vi "State Callers.vi"(8 "synchronization":refnum<class "synchronization.lvclass">, 9 "Callers":T2, 10 "State":string, 11 "Calling VI Details":T1) -> (0 "error out":errorcluster)   [LabVIEW 2020]
uses:
  JKI State Machine API/source/Support/State Calls Array.ctl
  JKI State Machine API/source/Support/State Call Cluster.ctl
  JKI State Machine API/source/JKI SM/JKI SM.lvclass/JKI SM.ctl
  <userlib>/_OpenG.lib/error/error.llb/Filter Error Codes (Array)__ogtk.vi
  <vilib>/regexp/Match Regular Expression.xnode
  JKI State Machine API/source/JKI SM/JKI SM.lvclass
  <userlib>/_OpenG.lib/error/error.llb/openg_error.lvlib
  synchronization/synchronization.lvclass
panel:
  in  "Listbox":i32(listbox)
  in  "OK":bool
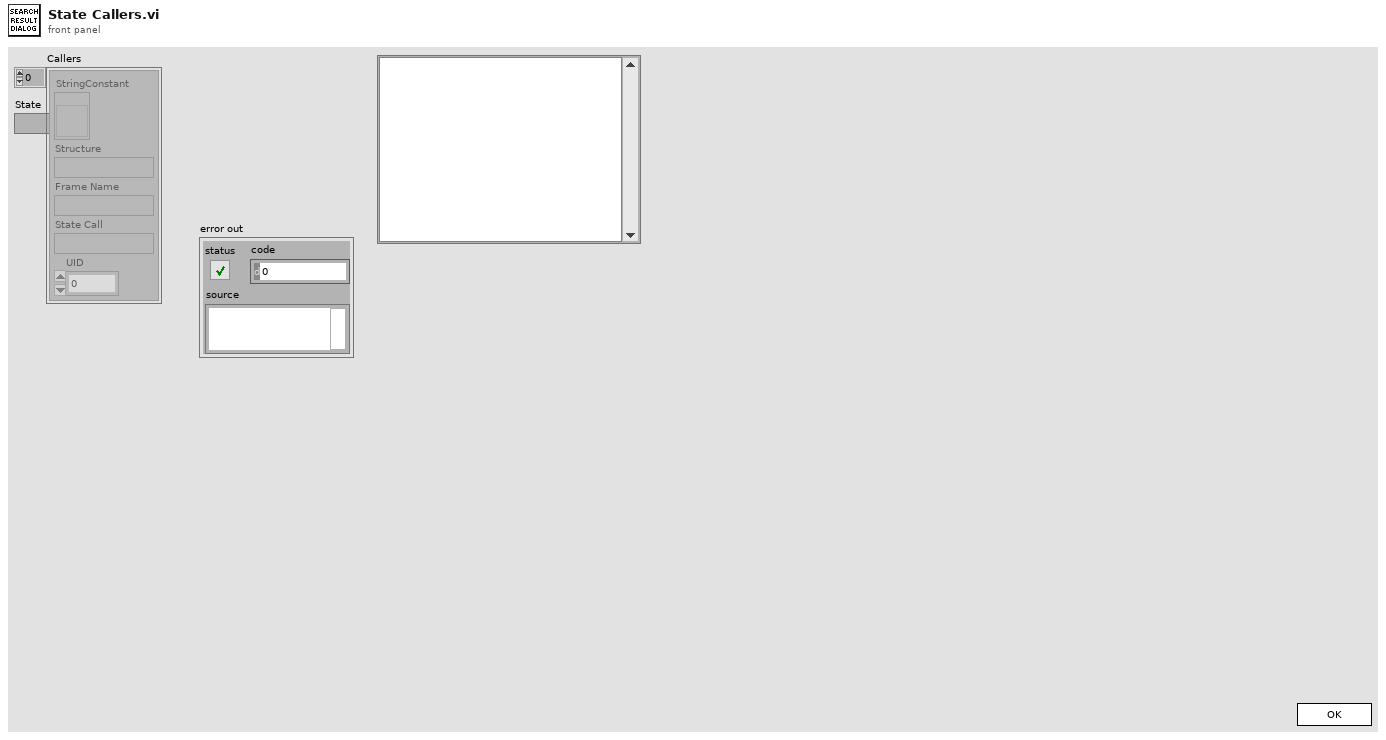
[diagram p1: front panel]
types:
  T1 = cluster{"App.ContextName":string, "VI.Name":string, "Object UID":i32}
  T2 = typedef "State Calls Array.ctl" = T3[]
  T3 = typedef "State Call Cluster.ctl" = cluster{"StringConstant":refnum<vi>, "Structure":string, "Frame Name":string, "State Call":string, "UID":i32}
  T4 = enum32{"Invalid", "Standard", "Closed", "Hidden", "Minimized", "Maximized"}
  T5 = enum32{"invalid app kind", "Development System", "Run Time System", "Student Edition", "Embedded LabVIEW", "Evaluation", "Custom"}
  T6 = enum32{"Invalid", "Default", "Floating", "Floating/Auto-Hide", "Modal"}
  T7 = cluster{"Core":cluster{"Current VI Reference":refnum<vi>, "Close Panel on Exit?":bool}, "Your Boolean data":bool, "Your string data":string, "State":string, "JKI SM out":refnum<class "JKI SM.lvclass">, "Callers":T2, "Application":refnum<vi>, "Owning VI":refnum<vi>}
  T8 = typedef "LVPoint32TypeDef.ctl" = cluster{"Horizontal":i32, "Vertical":i32}
  T9 = cluster{"Shift":bool, "Ctrl":bool, "Alt":bool, "Cmd":bool, "Opt":bool}
  T10 = cluster{"StringConstant":refnum<vi>, "Structure":string, "Frame Name":string, "State Call":string, "UID":dbl}[]
  T11 = cluster{"Current VI Reference":refnum<vi>, "Close Panel on Exit?":bool}
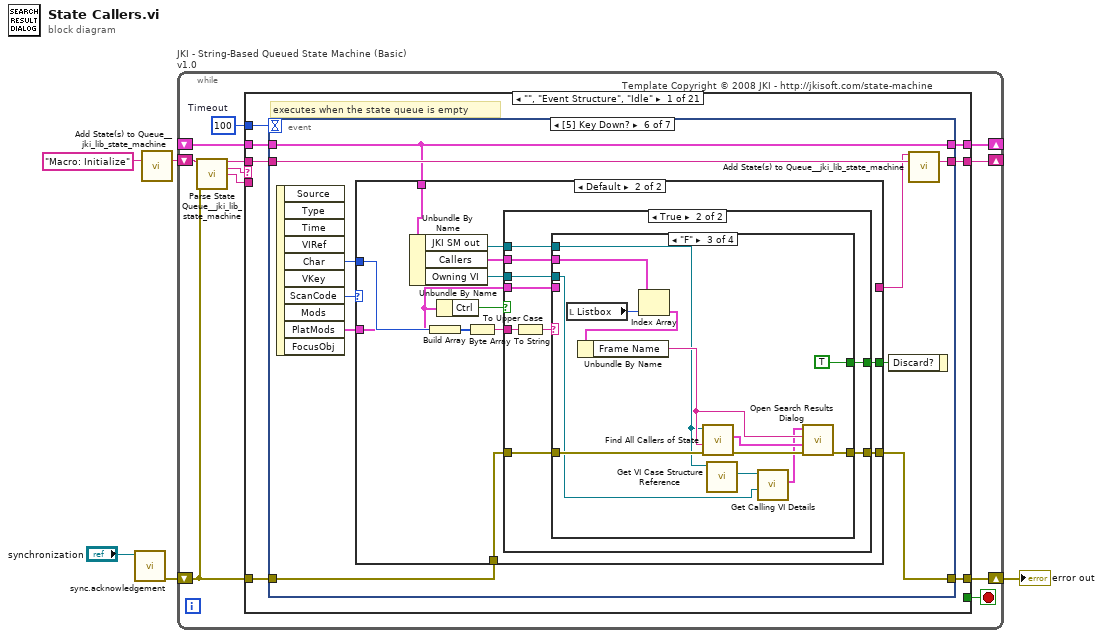
[diagram p0: block diagram]
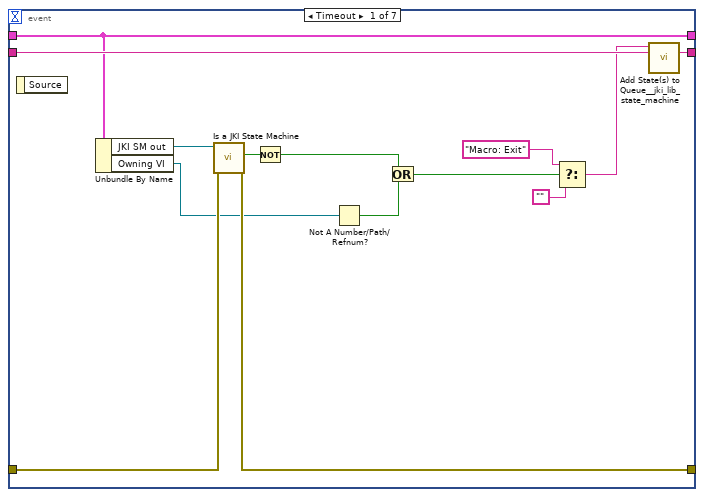
[diagram p2: hidden frame]
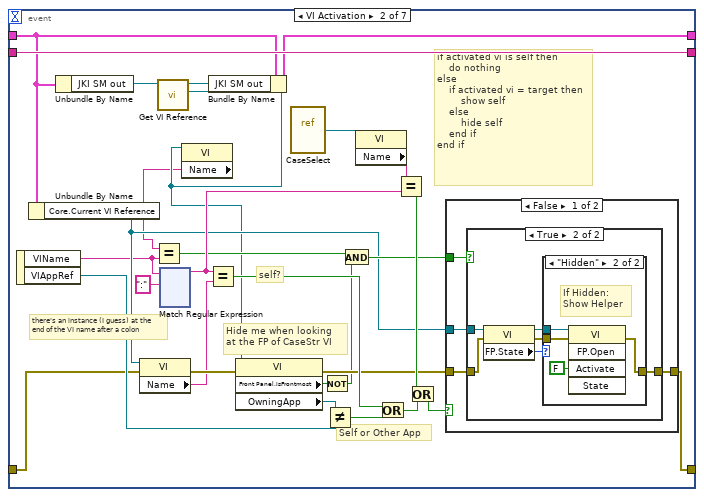
[diagram p3: hidden frame]
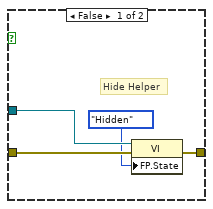
[diagram p4: hidden frame]
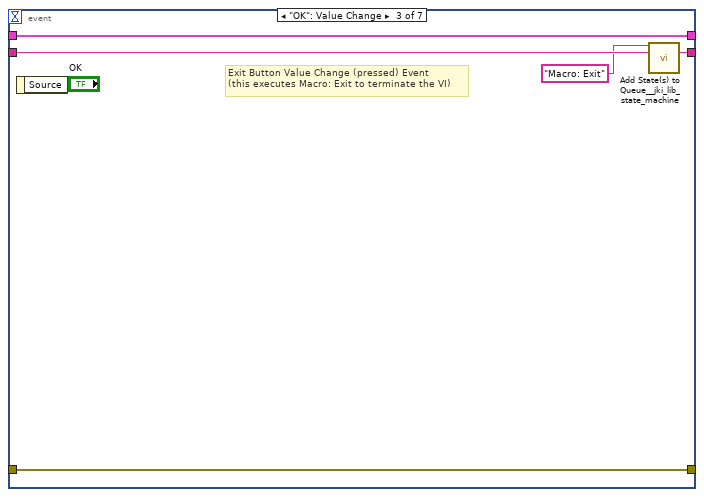
[diagram p7: hidden frame]
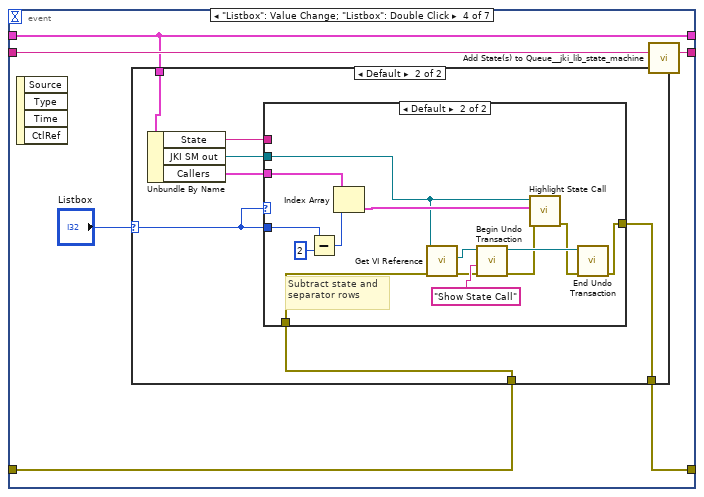
[diagram p8: hidden frame]
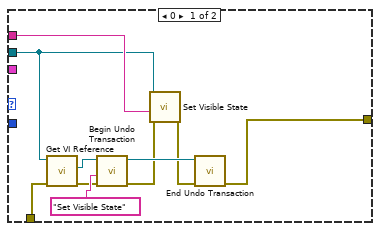
[diagram p10: hidden frame]
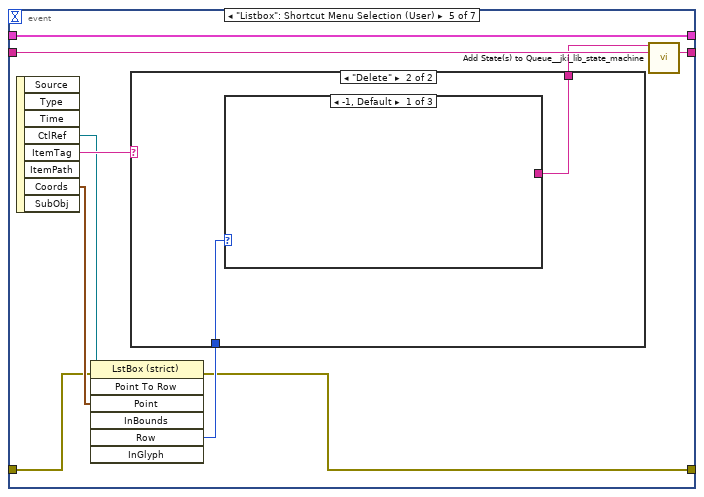
[diagram p11: hidden frame]
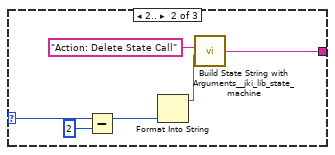
[diagram p13: hidden frame]
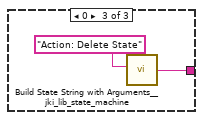
[diagram p14: hidden frame]
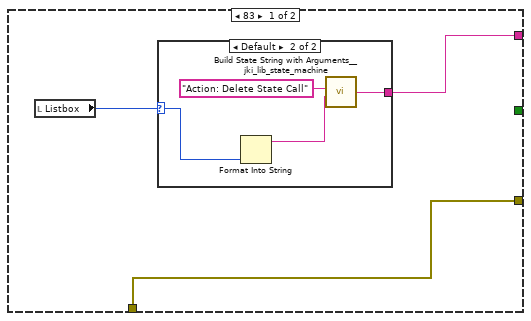
[diagram p15: hidden frame]
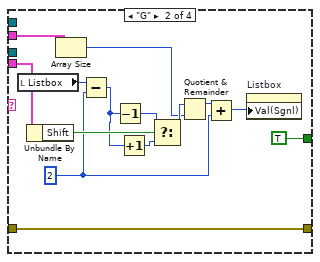
[diagram p19: hidden frame]
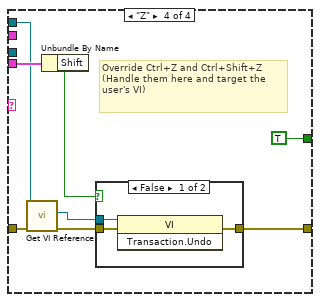
[diagram p20: hidden frame]
diagram:
  n1 = call "sync.acknowledgement.vi"("synchronization"="synchronization") -> ("error out"=w2:errorcluster)  [unwired: 10 in]
  n2 = call <vilib>:"Add State(s) to Queue__jki_lib_state_machine.vi"("State(s) in (\"\")"="Macro: Initialize") -> ("States Out"=w5:string)  [unwired: 14 in]
  n3 = while "JKI - String-Based Queued State Machine (Basic) v1.0" {
    shift-right: [w9] -> _
    shift-left: _ -> [w8]
    shift-right: [w12] -> w3
    shift-left: w2 -> [w6]
    shift-right: [w11] -> _
    shift-left: w5 -> [w13]
    stop <- w10 stop-if-true
    w7 = 100  # Timeout
    # "Template Copyright © 2008 JKI - http://jkisoft.com/state-machine"
    n4 = call <vilib>:"Parse State Queue__jki_lib_state_machine.vi"("State Queue"=w13, "Error In (no error)"=w6) -> ("Remaining States"=w15:string, "Current State"=w16:string, "Arguments"=w14:string)  [unwired: 11 in]
    n5 = case shown="\"\", \"Event Structure\", \"Idle\"" w16 {
      selector: w16 -> [_ _ w352 _ _ _ _ _ _ _ _ _ _ _ _ _ _ _ _ _ _]
      tunnel: w15 -> [w23 w351 w356 w376 w387 w392 w396 w418 w442 w448 w466 w481 w499 w510 w539 w544 w554 w558 w568 w600 w632]
      tunnel: w14 -> [_ _ _ _ _ _ _ _ _ _ _ _ w494 w504 _ _ _ _ w566 _ _]
      tunnel: w8 -> [w21 w348 w354 w368 w384 w390 w393 _ w439 w445 w463 w475 w497 w506 w536 w542 w551 w555 w560 w608 w629]
      tunnel: [w20 w349 w358 w363 errorcluster {"status"=FALSE, "code"=0, "source"=""} ("error out") w389 w394 w402 w435 w446 w464 w472 w495 w507 w537 w540 w552 w556 w561 w611 w630] -> w12
      tunnel: w6 -> [w19 w349 w357 w364 w382 w389 w394 w405 w430 w446 w464 w473 w496 w508 w537 w540 w552 w556 w564 w612 w630]
      tunnel: [w22 w350 w355 w375 w386 w391 w395 w417 w441 w447 w465 w480 w498 w509 w538 w543 w553 w557 w567 w613 w631] -> w11
      tunnel: [_ _ _ _ _ TRUE _ _ _ _ _ _ _ _ _ _ _ _ _ _ _] -> w10
      tunnel: [w18 w348 w354 w374 w384 w390 w393 w416 w439 w445 w463 w475 w497 w506 w536 w542 w551 w555 w559 w610 w629] -> w9
      tunnel: w7 -> [w17 _ _ _ _ _ _ _ _ _ _ _ _ _ _ _ _ _ _ _ _]
      frame "", "Event Structure", "Idle" {
        # "executes when the state queue is empty"
        n6 = event shown="[5] Key Down?" {
          selector: _ -> [_ _ _ _ _ _ _]
          dyn-events: _ -> [_ _ _ _ _ _ _]
          timeout: w17 -> [_ _ _ _ _ _ _]
          tunnel: w23 -> [w37 w66 w202 w208 w250 w270 w347]
          tunnel: [w36 w66 w201 w207 w249 w269 w346] -> w22
          tunnel: w21 -> [w32 w40 w199 w206 w242 w268 w344]
          tunnel: [w27 w41 w200 w204 w241 w263 w345] -> w20
          tunnel: w19 -> [w28 w42 w200 w205 w244 w264 w345]
          tunnel: [w32 w39 w199 w206 w242 w268 w344] -> w18
          event Timeout {
            n7 = event-data() -> ()  [unwired: 1 in, 1 out]
            n8 = Unbundle By Name(w32) -> ("JKI SM out"=w31:refnum<class "JKI SM.lvclass">, "Owning VI"=w24:refnum<vi>)
            n9 = call "Is a JKI State Machine.vi"("error in (no error)"=w28, "JKI SM in"=w31) -> ("error out"=w27:errorcluster, "Is a JKI State Machine"=w30:bool)  [unwired: 7 in, 1 out]
            n10 = Not(x=w30) -> (.not. x?=w29:bool)
            n11 = Not A Number/Path/Refnum?(number/path/refnum=w24) -> (NaN/Path/Refnum?=w26:bool)
            n12 = Or(x=w29, y=w26) -> (x .or. y?=w25:bool)
            n13 = Select(t="Macro: Exit", s=w25, f="") -> (s? t:f=w33:string)
            n14 = call <vilib>:"Add State(s) to Queue__jki_lib_state_machine.vi"("State(s) in Front (\"\")"=w33, "State(s) in (\"\")"=w37) -> ("States Out"=w36:string)  [unwired: 13 in]
          }
          event VI Activation {
            # "Self or Other App"
            # "self?"
            # "Hide me when looking\nat the FP of CaseStr VI"
            # "there's an instance (I guess) at the\nend of the VI name after a colon"
            # "if activated vi is self then\n    do nothing\nelse\n    if activated vi = target then\n        show self\n    else\n        hide self\n    end if\nend if"
            n15 = event-data() -> ("VIName"=w44:string, "VIAppRef"=w43:refnum<vi>)  [unwired: 1 in]
            n16 = Unbundle By Name(w40) -> ("Core.Current VI Reference"=w51:refnum<vi>)
            n17 = Unbundle By Name(w40) -> ("JKI SM out"=w47:refnum<class "JKI SM.lvclass">)
            n18 = property class="VI"(reference=w51, error in=w42) -> (error out=w55:errorcluster, "Name"=w50:string)  [unwired: 1 out]
            n19 = call "Get VI Reference.vi"("JKI SM in"=w47) -> ("VI"=w46:refnum<vi>, "JKI SM out"=w38:refnum<class "JKI SM.lvclass">)  [unwired: 8 in, 1 out]
            n20 = xnode "Match Regular Expression"("input string"=w44, "regular expression"=":") -> ("before match"=w62:string)  [unwired: 3 in, 5 out]
            n21 = property class="VI"(reference=w46) -> ("Name"=w45:string)  [unwired: 1 in, 2 out]
            n22 = Equal?(x=w45, y=w44) -> (x = y?=w48:bool)
            n23 = Equal?(x=w62, y=w50) -> (x = y?=w59:bool)
            n24 = Bundle By Name(cluster=w40, "JKI SM out"=w38) -> (w39:T7)
            n25 = property class="VI"(reference=w46, error in=w55) -> (error out=w54:errorcluster, "Front Panel.IsFrontmost"=w52:bool, "OwningApp"=w57:refnum<vi>)  [unwired: 1 out]
            n26 = vi-ref "CaseSelect.vi"() -> (w60:refnum<vi>)
            n27 = Not(x=w52) -> (.not. x?=w53:bool)
            n28 = Not Equal?(x=w57, y=w43) -> (x != y?=w58:bool)
            n29 = And(x=w48, y=w53) -> (x .and. y?=w56:bool)
            n30 = property class="VI"(reference=w60) -> ("Name"=w61:string)  [unwired: 1 in, 2 out]
            n31 = Or(x=w59, y=w58) -> (x .or. y?=w64:bool)
            n32 = Equal?(x=w61, y=w62) -> (x = y?=w63:bool)
            n33 = Or(x=w63, y=w64) -> (x .or. y?=w65:bool)
            n34 = case shown="False" w65 {
              tunnel: w54 -> [w70 w86]
              tunnel: [w68 w86] -> w41
              tunnel: w51 -> [w69 _]
              tunnel: w56 -> [w67 _]
              frame False {
                n35 = case shown="True" w67 {
                  tunnel: w70 -> [w74 w79]
                  tunnel: w69 -> [w73 w80]
                  tunnel: [w72 w77] -> w68
                  frame False {
                    # "Hide Helper"
                    n36 = property class="VI"(reference=w73, error in=w74, "FP.State"=T4."Hidden" ("Front Panel Window:State")) -> (error out=w72:errorcluster)  [unwired: 1 out]
                  }
                  frame True {
                    n37 = property class="VI"(reference=w80, error in=w79) -> (reference out=w76:refnum<vi>, error out=w75:errorcluster, "FP.State"=w78:T4)
                    n38 = case shown="\"Hidden\"" w78 {
                      tunnel: [w81 w85] -> w77
                      tunnel: w76 -> [_ w84]
                      tunnel: w75 -> [w81 w83]
                      frame Default {
                      }
                      frame "Hidden" {
                        # "If Hidden:\nShow Helper"
                        n39 = invoke class="VI" method="FP.Open"(reference=w84, error in=w83, "Activate"=FALSE ("Activate?")) -> (error out=w85:errorcluster)  [unwired: 2 in, 4 out]
                      }
                    }
                  }
                }
              }
              frame True {
              }
            }
          }
          event "OK": Value Change {
            # "Exit Button Value Change (pressed) Event\n(this executes Macro: Exit to terminate the VI)"
            n40 = event-data() -> ()  [unwired: 1 in, 1 out]
            n41 = call <vilib>:"Add State(s) to Queue__jki_lib_state_machine.vi"("State(s) in Front (\"\")"="Macro: Exit", "State(s) in (\"\")"=w202) -> ("States Out"=w201:string)  [unwired: 13 in]
          }
          event "Listbox": Value Change; "Listbox": Double Click {
            n42 = event-data() -> ()  [unwired: 1 in, 4 out]
            n43 = case shown="Default" "Listbox" {
              selector: "Listbox" -> [_ w210]
              tunnel: w206 -> [_ w216]
              tunnel: w205 -> [w209 w213]
              tunnel: [w209 w212] -> w204
              frame -1 {
              }
              frame Default {
                n44 = Unbundle By Name(w216) -> ("State"=w211:string, "JKI SM out"=w214:refnum<class "JKI SM.lvclass">, "Callers"=w215:T2)
                n45 = case shown="Default" w210 {
                  tunnel: w215 -> [_ w240]
                  tunnel: w214 -> [w220 w232]
                  tunnel: w213 -> [w221 w228]
                  tunnel: w210 -> [_ w237]
                  tunnel: [w217 w229] -> w212
                  tunnel: w211 -> [w226 _]
                  frame 0 {
                    n46 = call "Get VI Reference.vi"("error in (no error)"=w221, "JKI SM in"=w220) -> ("error out"=w224:errorcluster, "VI"=w223:refnum<vi>)  [unwired: 7 in, 1 out]
                    n47 = call "Begin Undo Transaction.vi"("error in (no error)"=w224, "Action"="Set Visible State", "VI in"=w223) -> ("error out"=w219:errorcluster, "VI out"=w222:refnum<vi>)  [unwired: 7 in]
                    n48 = call "Set Visible State.vi"("error in (no error)"=w219, "State Name"=w226, "JKI SM in"=w220) -> ("error out"=w218:errorcluster)  [unwired: 7 in, 1 out]
                    n49 = call "End Undo Transaction.vi"("error in (no error)"=w218, "VI in"=w222) -> ("error out"=w217:errorcluster)  [unwired: 8 in, 1 out]
                  }
                  frame Default {
                    # "Subtract state and separator rows"
                    n50 = Subtract(x=w237, y=2) -> (x-y=w236:i32)
                    n51 = Index Array(array=w240, index=w236) -> (element=w239:T3)
                    n52 = call "Get VI Reference.vi"("error in (no error)"=w228, "JKI SM in"=w232) -> ("error out"=w234:errorcluster, "VI"=w233:refnum<vi>)  [unwired: 7 in, 1 out]
                    n53 = call "Begin Undo Transaction.vi"("error in (no error)"=w234, "Action"="Show State Call", "VI in"=w233) -> ("error out"=w227:errorcluster, "VI out"=w231:refnum<vi>)  [unwired: 7 in]
                    n54 = call "Highlight State Call.vi"("error in (no error)"=w227, "State Call"=w239, "JKI SM in"=w232) -> ("error out"=w230:errorcluster)  [unwired: 7 in, 1 out]
                    n55 = call "End Undo Transaction.vi"("error in (no error)"=w230, "VI in"=w231) -> ("error out"=w229:errorcluster)  [unwired: 8 in, 1 out]
                  }
                }
              }
            }
            n56 = call <vilib>:"Add State(s) to Queue__jki_lib_state_machine.vi"("State(s) in (\"\")"=w208) -> ("States Out"=w207:string)  [unwired: 14 in]
          }
          event "Listbox": Shortcut Menu Selection (User) {
            n57 = event-data() -> ("CtlRef"=w247:refnum<vi>, "ItemTag"=w248:string, "Coords"=w246:T8)  [unwired: 1 in, 5 out]
            n58 = invoke class="LstBox (strict)" method="Point To Row"(reference=w247, error in=w244, "Point"=w246) -> (error out=w241:errorcluster, "Row"=w245:i32)  [unwired: 4 in, 5 out]
            n59 = case shown="\"Delete\"" w248 {
              tunnel: w245 -> [_ w252]
              tunnel: [_ w251] -> w243
              frame Default {
              }
              frame "Delete" {
                n60 = case shown="-1, Default" w252 {
                  selector: w252 -> [_ w255 _]
                  tunnel: [_ w256 w259] -> w251
                  frame -1, Default {
                  }
                  frame 2.. {
                    n61 = Subtract(x=w255, y=2) -> (x-y=w254:i32)
                    n62 = Format Into String(w254) -> (resulting string=w257:string)  [unwired: 3 in, 1 out]
                    n63 = call <vilib>:"Build State String with Arguments__jki_lib_state_machine.vi"("Arguments (\"\")"=w257, "State"="Action: Delete State Call") -> ("State with Arguments"=w256:string)  [unwired: 4 in]
                  }
                  frame 0 {
                    n64 = call <vilib>:"Build State String with Arguments__jki_lib_state_machine.vi"("State"="Action: Delete State") -> ("State with Arguments"=w259:string)  [unwired: 5 in]
                  }
                }
              }
            }
            n65 = call <vilib>:"Add State(s) to Queue__jki_lib_state_machine.vi"("State(s) in Front (\"\")"=w243, "State(s) in (\"\")"=w250) -> ("States Out"=w249:string)  [unwired: 13 in]
          }
          event Key Down? {
            n66 = event-data() -> ("Char"=w267:i16, "ScanCode"=w262:i16, "PlatMods"=w266:T9)  [unwired: 1 in, 7 out]
            n67 = case shown="Default" w262 {
              tunnel: w268 -> [_ w289]
              tunnel: w267 -> [_ w287]
              tunnel: w266 -> [_ w284]
              tunnel: [_ w282] -> w265
              tunnel: w264 -> [w272 w280]
              tunnel: [w272 w279] -> w263
              tunnel: [w271 _] -> w261
              frame 83 {
                n68 = local read "Listbox"() -> (w273:i32)
                n69 = case shown="Default" w273 {
                  selector: w273 -> [_ w274]
                  tunnel: [_ w275] -> w271
                  frame -1 {
                  }
                  frame Default {
                    n70 = Format Into String(w274) -> (resulting string=w276:string)  [unwired: 3 in, 1 out]
                    n71 = call <vilib>:"Build State String with Arguments__jki_lib_state_machine.vi"("Arguments (\"\")"=w276, "State"="Action: Delete State Call") -> ("State with Arguments"=w275:string)  [unwired: 4 in]
                  }
                }
              }
              frame Default {
                n72 = Unbundle By Name(w289) -> ("JKI SM out"=w281:refnum<class "JKI SM.lvclass">, "Callers"=w288:T2, "Owning VI"=w278:refnum<vi>)
                n73 = Build Array(w287) -> (w286:i16[])
                n74 = Unbundle By Name(w284) -> ("Ctrl"=w283:bool)
                n75 = Byte Array To String(unsigned byte array=w286) -> (string=w285:string)
                n76 = case shown="True" w283 {
                  tunnel: w288 -> [_ w299]
                  tunnel: w285 -> [_ w298]
                  tunnel: w284 -> [_ w297]
                  tunnel: [_ w296] -> w282
                  tunnel: w281 -> [_ w294]
                  tunnel: [w290 w293] -> w279
                  tunnel: w280 -> [w290 w292]
                  tunnel: w278 -> [_ w291]
                  frame False {
                  }
                  frame True {
                    n77 = To Upper Case(1:w298) -> (0:w295:string)
                    n78 = case shown="\"F\"" w295 {
                      tunnel: w299 -> [_ w314 w325 _]
                      tunnel: w297 -> [_ w309 _ w334]
                      tunnel: [_ TRUE TRUE TRUE] -> w296
                      tunnel: w294 -> [_ _ w318 w331]
                      tunnel: [w300 w307 w319 w328] -> w293
                      tunnel: w292 -> [w300 w307 w320 w332]
                      tunnel: w291 -> [_ _ w315 _]
                      frame Default {
                      }
                      frame "G" {
                        w302 = 2 ("y")
                        n79 = local read "Listbox"() -> (w304:i32)
                        n80 = Unbundle By Name(w309) -> ("Shift"=w310:bool)
                        n81 = Array Size(array=w314) -> (size(s)=w301:i32)
                        n82 = Subtract(x=w304, y=w302) -> (x-y=w303:i32)
                        n83 = Decrement(x=w303) -> (x-1=w312:i32)
                        n84 = Increment(x=w303) -> (x+1=w313:i32)
                        n85 = Select(t=w312, s=w310, f=w313) -> (s? t:f=w311:i32)
                        n86 = Quotient & Remainder(x=w311, y=w301) -> (x-y*floor(x/y)=w306:i32)  [unwired: 1 out]
                        n87 = Add(x=w306, y=w302) -> (x+y=w305:i32)
                        n88 = property on="Listbox" class="LstBox (strict)"("Val(Sgnl)"=w305) -> ()  [unwired: 2 in, 2 out]
                      }
                      frame "F" {
                        n89 = local read "Listbox"() -> (w326:i32)
                        n90 = Index Array(array=w325, index=w326) -> (element=w324:T3)
                        n91 = Unbundle By Name(w324) -> ("Frame Name"=w321:string)
                        n92 = call "Find All Callers of State.vi"("error in (no error)"=w320, "State Name"=w321, "JKI SM in"=w318) -> ("error out"=w322:errorcluster, "Callers"=w323:T10)  [unwired: 6 in, 1 out]
                        n93 = call "Get VI Case Structure Reference.vi"("JKI SM in"=w318) -> ("Case Structure ref"=w317:refnum<vi>)  [unwired: 8 in, 2 out]
                        n94 = call "Get Calling VI Details.vi"("User VI Ref"=w315, "Affected Items"=w317) -> ("Calling VI Details"=w316:T1)  [unwired: 9 in]
                        n95 = call "Open Search Results Dialog.vi"("error in (no error)"=w322, "Callers"=w323, "State"=w321, "Calling VI Details"=w316) -> ("error out"=w319:errorcluster)  [unwired: 7 in]
                      }
                      frame "Z" {
                        # "Override Ctrl+Z and Ctrl+Shift+Z\n(Handle them here and target the user's VI)"
                        n96 = call "Get VI Reference.vi"("error in (no error)"=w332, "JKI SM in"=w331) -> ("error out"=w329:errorcluster, "VI"=w330:refnum<vi>)  [unwired: 7 in, 1 out]
                        n97 = Unbundle By Name(w334) -> ("Shift"=w333:bool)
                        n98 = case shown="False" w333 {
                          tunnel: w330 -> [w338 w341]
                          tunnel: w329 -> [w336 w340]
                          tunnel: [w337 w339] -> w328
                          frame False {
                            n99 = invoke class="VI" method="Transaction.Undo"(reference=w338, error in=w336) -> (error out=w337:errorcluster)  [unwired: 1 in, 2 out]
                          }
                          frame True {
                            n100 = invoke class="VI" method="Transaction.Redo"(reference=w341, error in=w340) -> (error out=w339:errorcluster)  [unwired: 1 in, 2 out]
                          }
                        }
                      }
                    }
                  }
                }
              }
            }
            n101 = event-data("Discard?"=w265) -> ()  [unwired: 1 in, 1 out]
            n102 = call <vilib>:"Add State(s) to Queue__jki_lib_state_machine.vi"("State(s) in Front (\"\")"=w261, "State(s) in (\"\")"=w270) -> ("States Out"=w269:string)  [unwired: 13 in]
          }
          event Panel Close? {
            # "Discard the event because we'll close the front panel ourselves in Macro: Exit"
            # "Close Panel button (pressed) Event\n(this executes Macro: Exit to terminate the VI)"
            n103 = event-data() -> ()  [unwired: 1 in, 1 out]
            n104 = event-data("Discard?"=TRUE) -> ()  [unwired: 1 in, 1 out]
            n105 = call <vilib>:"Add State(s) to Queue__jki_lib_state_machine.vi"("State(s) in Front (\"\")"="Macro: Exit", "State(s) in (\"\")"=w347) -> ("States Out"=w346:string)  [unwired: 13 in]
          }
        }
      }
      frame "---------- Core ----------" {
        # "Do not put any code in this frame.\n(it is a separator no-op)"
        n106 = call <vilib>:"Add State(s) to Queue__jki_lib_state_machine.vi"("State(s) in (\"\")"=w351) -> ("States Out"=w350:string)  [unwired: 14 in]
      }
      frame Default {
        w361 = 42 items=["No error", "Argument error", "Memory is full", "Out of zone", "End of file", "File already open", "Generic file I/O error", "File not found", "File permission error", "Disk is full", "Duplicate path", "Too many files open", "System feature not enabled", "Resource file not found", "Cannot add resource", "Resource not found", "Image not found", "Image memory error", "Pen does not exist", "Config type invalid", "Config token not found", "Config parse error", "Config memory error", "Bad external code format", "Bad external code offset", "External code not present", "Null window", "Destroy window error", "Null menu", "Print aborted", "Bad print record", "Print driver error", "Windows error during printing", "Memory error during printing", "Print dialog error", "Generic print error", "Invalid device refnum", "Device not found", "Device parameter error", "Device unit error", "Cannot open device", "Device call aborted", "Generic error", "Cancelled by user", "Object ID too low", "Object ID too high", "Object not in heap", "Unknown heap", "Unknown object (invalid DefProc)", "Unknown object (DefProc not in table)", "Message out of range", "Invalid (null) method", "Unknown message", "Manager call not supported", "Bad address", "Network operation in progress", "Network operation timed out", "Connection is busy", "Network attribute not supported", "Network error", "Address in use", "System out of memory", "Connection aborted", "Connection refused", "Not connected", "Already connected", "Connection closed", "Initialization error (interapplication manager)", "Bad occurrence", "Wait on unbound occurrence handler", "Occurrence queue overflow", "Datalog type conflict", "Unused", "Unrecognized type (interapplication manager)", "Memory corrupt", "Failed to make temporary DLL", "Old CIN version", "Drag socket not found", "Failed to load drop-object", "Failed to register OLE object", "Failed to release OLE object", "Format specifier type mismatch", "Unknown format specifier", "Too few format specifiers", "Too many format specifiers", "Scan failed", "Newer CIN version", "Error converting to variant", "Runtime menu error", "Password tampered", "Variant attribute not found", "Incompatible variant data type", "Event data is not available", "Event Store is not present", "Occurrence is not found", "Event Queue is not created", "Event info is not available", "Refnum passed is NULL", "Error retrieving Class GUID", "Error retrieving CoClass GUID", "Error retrieving TypeLib GUID.", "Bad built application magic bytes.", "Specific driver is different from the specific driver associated with the Logical Name.", "There is no session opened to the class driver.", "Max Error", "MAX - Error with config objects", "MAX - Error loading configuration", "MAX - Group not supported"]
        # "Current State"
        # "Do not delete, rename, or modify this frame.\n(this is used to capture unhandled states and typos)"
        # "Handle mistyped state name (developer tool)"
        n107 = Format Into String(format string="Software Exception: Unhandled State \"%s\"." ("message"), error in=w357, w352) -> (resulting string=w360:string, error out=w359:errorcluster)  [unwired: 1 in]
        n108 = call <vilib>:"Error Cluster From Error Code.vi"("show call chain? (False)"=TRUE, "error in (no error)"=w359, "error message (\"\")"=w360, "error code (0)"=w361) -> ("error out"=w358:errorcluster)  [unwired: 5 in]
        n109 = call <vilib>:"Add State(s) to Queue__jki_lib_state_machine.vi"("State(s) in (\"\")"=w356) -> ("States Out"=w355:string)  [unwired: 14 in]
      }
      frame "Initialize Core Data" {
        # "Do not delete, rename, or modify this frame.\n(this is used to determine panel behavior on exit)"
        # "originally closed?"
        # "exe?"
        # "If panel starts closed or is an EXE, then close it when we exit"
        n110 = property class="VI"() -> ("Clone Name"=w366:string)  [unwired: 2 in, 2 out]
        n111 = Open VI Reference(vi path=w366, error in (no error)=w364) -> (vi reference=w365:refnum<vi>, error out=w363:errorcluster)  [unwired: 4 in]
        n112 = property class="VI"() -> ("Front Panel.Open"=w373:bool)  [unwired: 2 in, 2 out]
        n113 = property class="App"() -> ("App.Kind"=w372:T5)  [unwired: 2 in, 2 out]
        n114 = Not(x=w373) -> (.not. x?=w370:bool)
        n115 = Equal?(x=w372, y=T5."Run Time System" ("Application:Kind")) -> (x = y?=w369:bool)
        n116 = Or(x=w370, y=w369) -> (x .or. y?=w367:bool)
        n117 = Bundle By Name(cluster=w368, "Core.Current VI Reference"=w365, "Core.Close Panel on Exit?"=w367) -> (w374:T7)
        n118 = call <vilib>:"Add State(s) to Queue__jki_lib_state_machine.vi"("State(s) in (\"\")"=w376) -> ("States Out"=w375:string)  [unwired: 14 in]
      }
      frame "Error Handler" {
        w383 = i32[] [1026]  # JKI SM VI Invalid Ref
        # "Unhandled Error -- Display it"
        # "Handle any errors here.\nYou can also output any states to clean-up after errors occur"
        # "Clear error"
        n119 = call-poly <userlib>:"Filter Error Codes__ogtk.vi"("Error In"=w382, "Error Codes to Filter"=w383) -> ("Error Out"=w381:errorcluster, "Error Filtered?"=w380:bool)  [unwired: 7 in, 1 out]
        n120 = call <vilib>:"General Error Handler.vi"("error in (no error)"=w381) -> ()  [unwired: 10 in, 5 out]
        n121 = Select(t="Macro: Exit", s=w380, f="") -> (s? t:f=w377:string)
        n122 = call <vilib>:"Add State(s) to Queue__jki_lib_state_machine.vi"("State(s) in Front (\"\")"=w377, "State(s) in (\"\")"=w387) -> ("States Out"=w386:string)  [unwired: 13 in]
      }
      frame "Exit" {
        # "Do not put any code in this frame.\n(No errors that occur here will be handled.)"
        n123 = call <vilib>:"Add State(s) to Queue__jki_lib_state_machine.vi"("State(s) in (\"\")"=w392) -> ("States Out"=w391:string)  [unwired: 14 in]
      }
      frame "---------- Data ----------" {
        # "Do not put any code in this frame.\n(It is a separator no-op. You can make a copy of this frame to create a new Data frame)"
        n124 = call <vilib>:"Add State(s) to Queue__jki_lib_state_machine.vi"("State(s) in (\"\")"=w396) -> ("States Out"=w395:string)  [unwired: 14 in]
      }
      frame "Data: Initialize" {
        w413 = T11 {"Current VI Reference"=refnum, "Close Panel on Exit?"=FALSE}  # Core
        w415 = TRUE  # Your Boolean data
        w414 = ""  # Your string data
        # "do not delete - used by framework"
        # "Add new data here."
        # "Data names and types of shift register data are defined by this bundle."
        # "Initialize the shift-register data, here.\n(data names are defined by what you wire into the bundle function)"
        n125 = call "Get Affected Item.vi"("error in (no error)"=w405, "Owning VI Details"="Calling VI Details") -> ("error out"=w404:errorcluster, "GObject"=w409:refnum<vi>, "Owning VI"=w400:refnum<vi>, "Application"=w401:refnum<vi>)  [unwired: 6 in]
        n126 = To More Specific Class(target class=refnum<vi> refnum ("Structure"), reference=w409, error in=w404) -> (specific class reference=w407:refnum<vi>, error out=w406:errorcluster)
        n127 = call "Create (From Structure).vi"("error in (no error)"=w406, "Structure"=w407) -> ("error out"=w403:errorcluster, "JKI SM out"=w411:refnum<class "JKI SM.lvclass">)  [unwired: 8 in]
        n128 = for {
          tunnel: "Callers" -> [w428] mode=indexing
          tunnel: w400 -> [w427]
          tunnel: [w422] -> w399 mode=indexing
          shift-right: [w419] -> w402
          shift-left: w403 -> [w421]
          n129 = Unbundle By Name(w428) -> ("UID"=w426:i32)
          n130 = call <vilib>:"UID to GObject Reference.vi"("error in (no error)"=w421, "UID"=w426, "Owning VI"=w427) -> ("error out"=w420:errorcluster, "GObject"=w425:refnum<vi>)  [unwired: 6 in, 1 out]
          n131 = To More Specific Class(target class=refnum<vi> refnum ("StringConstant"), reference=w425, error in=w420) -> (specific class reference=w423:refnum<vi>, error out=w419:errorcluster)
          n132 = Bundle By Name(cluster=w428, "StringConstant"=w423) -> (w422:T3)
        }
        n133 = Coerce To Type(0:w399, 1:"Callers") -> (2:w398:T2)
        n134 = Bundle("Core"=w413, "Your Boolean data"=w415, "Your string data"=w414, "State"="State", "JKI SM out"=w411, "Callers"=w398, "Application"=w401, "Owning VI"=w400) -> (w416:T7)  [unwired: 1 in]
        n135 = call <vilib>:"Add State(s) to Queue__jki_lib_state_machine.vi"("State(s) in (\"\")"=w418) -> ("States Out"=w417:string)  [unwired: 14 in]
      }
      frame "Data: Cleanup" {
        # "Ignore Errors\n(e.g. reference already invalid)"
        # "Cleanup any data and references, here.\n(this is called automatically, by the Macro: Exit)"
        n136 = Unbundle By Name(w439) -> ("Core.Current VI Reference"=w440:refnum<vi>, "Callers"=w438:T2, "JKI SM out"=w432:refnum<class "JKI SM.lvclass">)
        n137 = for {
          tunnel: w438 -> [w444] mode=indexing
          tunnel: [w443] -> w437 mode=indexing
          n138 = Unbundle By Name(w444) -> ("StringConstant"=w443:refnum<vi>)
        }
        n139 = Close Reference(reference=w440, error in (no error)=w430) -> (error out=w436:errorcluster)
        n140 = Close Reference(reference=w437, error in (no error)=w430) -> (error out=w434:errorcluster)
        n141 = call "Destroy.vi"("error in (no error)"=w430, "JKI SM in"=w432) -> ("error out"=w431:errorcluster)  [unwired: 9 in]
        n142 = call <userlib>:"Clear All Errors__ogtk.vi"("Upsteam Error (optional)"=w430, "Error In"=w431) -> ("Error Out"=w429:errorcluster)  [unwired: 2 in]
        n143 = call <userlib>:"Clear All Errors__ogtk.vi"("Upsteam Error (optional)"=w430, "Error In"=w434) -> ("Error Out"=w433:errorcluster)  [unwired: 2 in]
        n144 = Merge Errors(w436, w433, w429) -> (w435:errorcluster)
        n145 = call <vilib>:"Add State(s) to Queue__jki_lib_state_machine.vi"("State(s) in (\"\")"=w442) -> ("States Out"=w441:string)  [unwired: 14 in]
      }
      frame "---------- UI ----------" {
        # "Do not put any code in this frame.\n(It is a separator no-op. You can make a copy of this frame to create a new UI frame)"
        n146 = call <vilib>:"Add State(s) to Queue__jki_lib_state_machine.vi"("State(s) in (\"\")"=w448) -> ("States Out"=w447:string)  [unwired: 14 in]
      }
      frame "UI: Initialize" {
        # "Initialize the User Interface, here.\n(this is called automatically, by the Macro: Init)"
        n147 = Unbundle By Name(w463) -> ("Core.Current VI Reference"=w461:refnum<vi>, "State"=w456:string, "Callers"=w462:T2)
        n148 = for {
          tunnel: w462 -> [w471] mode=indexing
          tunnel: [w468] -> w454 mode=indexing
          n149 = Unbundle By Name(w471) -> ("Structure"=w470:string, "Frame Name"=w469:string)
          n150 = Format Into String(format string="%s: %s", w470, w469) -> (resulting string=w468:string)  [unwired: 2 in, 1 out]
        }
        n151 = Format Into String(format string="Find Callers (%s)", w456) -> (resulting string=w459:string)  [unwired: 2 in, 1 out]
        n152 = property class="VI"(reference=w461, "Front Panel.Title"=w459) -> ()  [unwired: 1 in, 2 out]
        n153 = Build Array (concatenate)(w456, "" ("format string"), w454) -> (w455:string[])
        n154 = property on="Listbox" class="LstBox (strict)"("Item Names"=w455, "Value"=-1 ("Listbox")) -> (error out=w453:errorcluster, "Item Symbols"=w452:i32[])  [unwired: 2 in, 1 out]
        n155 = Replace Array Subset(array=w452, new element=-1 ("new element/subarray"), index=1) -> (w451:i32[])
        n156 = property on="Listbox" class="LstBox (strict)"(error in=w453, "Item Symbols"=w451) -> ()  [unwired: 1 in, 2 out]
        n157 = call <vilib>:"Add State(s) to Queue__jki_lib_state_machine.vi"("State(s) in (\"\")"=w466) -> ("States Out"=w465:string)  [unwired: 14 in]
      }
      frame "UI: Pre-Test for 0 or 1 Items" {
        n158 = Unbundle By Name(w475) -> ("JKI SM out"=w476:refnum<class "JKI SM.lvclass">, "State"=w478:string, "Callers"=w477:T2)
        n159 = Array Size(array=w477) -> (size(s)=w479:i32)
        n160 = case shown="1" w479 {
          tunnel: w478 -> [_ w487 _]
          tunnel: [_ "Macro: Exit" "Macro: Exit"] -> w474
          tunnel: w477 -> [_ _ w492]
          tunnel: w476 -> [_ _ w491]
          tunnel: w473 -> [w482 w483 w489]
          tunnel: [w482 w483 w488] -> w472
          frame Default {
          }
          frame 0 {
            n161 = Format Into String(format string="State %s has no callers.", w487) -> (resulting string=w485:string)  [unwired: 2 in, 1 out]
            n162 = One Button Dialog(message=w485) -> ()  [unwired: 1 in, 1 out]
          }
          frame 1 {
            n163 = Index Array(array=w492) -> (element=w490:T3)  [unwired: 1 in]
            n164 = call "Highlight State Call.vi"("error in (no error)"=w489, "State Call"=w490, "JKI SM in"=w491) -> ("error out"=w488:errorcluster)  [unwired: 7 in, 1 out]
          }
        }
        n165 = call <vilib>:"Add State(s) to Queue__jki_lib_state_machine.vi"("State(s) in Front (\"\")"=w474, "State(s) in (\"\")"=w481) -> ("States Out"=w480:string)  [unwired: 13 in]
      }
      frame "UI: Cursor Set" {
        # "Argument"
        # "Set and Unset Cursor Busy.\n(Usage: \"UI: Cursor Set >> Busy|Idle\")"
        n166 = case shown="\"Idle\", Default" w494 {
          tunnel: w496 -> [w501 w503]
          tunnel: [w500 w502] -> w495
          frame "Idle", Default {
            n167 = call <vilib>:"Unset Busy.vi"("error in (no error)"=w501) -> ("error out"=w500:errorcluster)  [unwired: 10 in]
          }
          frame "Busy" {
            n168 = call <vilib>:"Set Busy.vi"("error in (no error)"=w503) -> ("error out"=w502:errorcluster)  [unwired: 9 in, 1 out]
          }
        }
        n169 = call <vilib>:"Add State(s) to Queue__jki_lib_state_machine.vi"("State(s) in (\"\")"=w499) -> ("States Out"=w498:string)  [unwired: 14 in]
      }
      frame "UI: Front Panel State" {
        # "Argument"
        # "Set Front Panel Open or Closed\n(Usage: \"UI: Front Panel State >> Open|Close\")"
        n170 = Unbundle By Name(w506) -> ("Core.Current VI Reference"=w505:refnum<vi>)
        n171 = case shown="\"Open\", Default" w504 {
          tunnel: w508 -> [w514 w530]
          tunnel: [w516 w531] -> w507
          tunnel: w505 -> [w515 w528]
          frame "Open", Default {
            n172 = property class="VI"(reference=w515, error in=w514) -> (reference out=w512:refnum<vi>, error out=w513:errorcluster, "Front Panel.Open"=w511:bool)
            n173 = case shown="False" w511 {
              tunnel: [w519 w525] -> w516
              tunnel: w513 -> [w522 w525]
              tunnel: w512 -> [w521 _]
              frame False {
                # "Setting Floatin here, instead of VI Properties allows the VI to accept keyboard input immediately after openning. (setting it in VI Properties was causing a bug where it wouldn't receive keyboard input until clicking on the VI)"
                n174 = invoke class="VI" method="FP.Open"(reference=w521, error in=w522, "Activate"=TRUE, "State"=T4."Standard") -> (reference out=w518:refnum<vi>, error out=w520:errorcluster)  [unwired: 1 in, 3 out]
                n175 = property class="VI"(reference=w518, error in=w520, "FP.Behavior"=T6."Floating" ("Front Panel Window:Behavior")) -> (error out=w519:errorcluster)  [unwired: 1 out]
              }
              frame True {
              }
            }
          }
          frame "Close" {
            n176 = property class="VI"(reference=w528, error in=w530) -> (reference out=w527:refnum<vi>, error out=w529:errorcluster, "Front Panel.Open"=w526:bool)
            n177 = case shown="True" w526 {
              tunnel: [w532 w535] -> w531
              tunnel: w529 -> [w532 w534]
              tunnel: w527 -> [_ w533]
              frame False {
              }
              frame True {
                n178 = invoke class="VI" method="FP.Close"(reference=w533, error in=w534) -> (error out=w535:errorcluster)  [unwired: 1 in, 2 out]
              }
            }
          }
        }
        n179 = call <vilib>:"Add State(s) to Queue__jki_lib_state_machine.vi"("State(s) in (\"\")"=w510) -> ("States Out"=w509:string)  [unwired: 14 in]
      }
      frame "---------- Macro ----------" {
        # "Do not put any code in this frame.\n(It is a separator no-op. You can make a copy of this frame to create a new Macro frame)"
        n180 = call <vilib>:"Add State(s) to Queue__jki_lib_state_machine.vi"("State(s) in (\"\")"=w539) -> ("States Out"=w538:string)  [unwired: 14 in]
      }
      frame "Macro: Initialize" {
        w541 = "Data: Initialize\nInitialize Core Data\nUI: Pre-Test for 0 or 1 Items\nUI: Initialize\nUI: Front Panel State >> Open"  # Data: Initialize Initialize Core Data UI: Pre-Test for 0 or 1 Items UI: Initialize UI: Front Panel State >> Open
        # "Initialization Macro\n(This is called once, when the VI starts)"
        n181 = call <vilib>:"Add State(s) to Queue__jki_lib_state_machine.vi"("State(s) in Front (\"\")"=w541, "State(s) in (\"\")"=w544) -> ("States Out"=w543:string)  [unwired: 13 in]
      }
      frame "Macro: Exit" {
        # "Exit Macro\n(This is called once, when the VI exits)"
        n182 = Unbundle By Name(w551) -> ("Core.Close Panel on Exit?"=w550:bool)
        n183 = Select(t="UI: Front Panel State >> Close", s=w550, f="") -> (s? t:f=w547:string)
        n184 = call <vilib>:"Add State(s) to Queue__jki_lib_state_machine.vi"("State(s) in (\"\")"=w547, "State(s) at Back (\"\")"="Data: Cleanup\nExit") -> ("States Out"=w545:string)  [unwired: 13 in]
        n185 = call <vilib>:"Add State(s) to Queue__jki_lib_state_machine.vi"("State(s) in Front (\"\")"=w545, "State(s) in (\"\")"=w554) -> ("States Out"=w553:string)  [unwired: 13 in]
      }
      frame "---------- Action ----------" {
        # "Template Separator\n(You can make a copy of, or modify, this frame)"
        n186 = call <vilib>:"Add State(s) to Queue__jki_lib_state_machine.vi"("State(s) in (\"\")"=w558) -> ("States Out"=w557:string)  [unwired: 14 in]
      }
      frame "Action: Delete State Call" {
        n187 = Scan From String(format string="%d", input string=w566, error in=w564) -> (error out=w562:errorcluster, output 1=w563:i32)  [unwired: 2 in, 2 out]
        n188 = case shown="Default" w563 {
          selector: w563 -> [_ w581]
          tunnel: w560 -> [w569 w585]
          tunnel: w562 -> [w570 w576]
          tunnel: [w569 w584] -> w559
          tunnel: [w570 w572] -> w561
          frame -1 {
          }
          frame Default {
            n189 = Unbundle By Name(w585) -> ("JKI SM out"=w586:refnum<class "JKI SM.lvclass">, "Callers"=w582:T2, "JKI SM out"=w578:refnum<class "JKI SM.lvclass">)
            n190 = call "Get VI Reference.vi"("error in (no error)"=w576, "JKI SM in"=w578) -> ("error out"=w575:errorcluster, "VI"=w577:refnum<vi>)  [unwired: 7 in, 1 out]
            n191 = call "Begin Undo Transaction.vi"("error in (no error)"=w575, "Action"="Delete State Call", "VI in"=w577) -> ("error out"=w579:errorcluster, "VI out"=w573:refnum<vi>)  [unwired: 7 in]
            n192 = Index Array(array=w582, index=w581) -> (element=w580:T3)
            n193 = call "Delete State Call.vi"("error in (no error)"=w579, "State Call"=w580, "JKI SM in"=w586) -> ("error out"=w583:errorcluster)  [unwired: 7 in, 1 out]
            n194 = case shown="No Error" w583 {
              tunnel: w583 -> [w597 w598]
              tunnel: w581 -> [w589 _]
              tunnel: w585 -> [w593 w599]
              tunnel: [w592 w599] -> w584
              tunnel: w582 -> [w591 _]
              tunnel: [w587 w598] -> w571
              frame No Error {
                n195 = property on="Listbox" class="LstBox (strict)"(error in=w597) -> (error out=w596:errorcluster, "Item Names"=w595:string[])  [unwired: 1 in, 1 out]
                n196 = Delete From Array(array=w591, index=w589) -> (array with subset deleted=w590:T2)  [unwired: 1 in, 1 out]
                n197 = Bundle By Name(cluster=w593, "Callers"=w590) -> (w592:T7)
                n198 = Delete From Array(array=w595, index=w589) -> (array with subset deleted=w594:string[])  [unwired: 1 in, 1 out]
                n199 = property on="Listbox" class="LstBox (strict)"(error in=w596, "Item Names"=w594, "Value"=-1 ("Listbox")) -> (error out=w587:errorcluster)  [unwired: 1 in, 1 out]
              }
              frame Error {
              }
            }
            n200 = call "End Undo Transaction.vi"("error in (no error)"=w571, "VI in"=w573) -> ("error out"=w572:errorcluster)  [unwired: 8 in, 1 out]
          }
        }
        n201 = call <vilib>:"Add State(s) to Queue__jki_lib_state_machine.vi"("State(s) in (\"\")"=w568) -> ("States Out"=w567:string)  [unwired: 14 in]
      }
      frame "Action: Delete State" {
        n202 = Unbundle By Name(w608) -> ("State"=w606:string, "Callers"=w607:T2)
        n203 = Array Size(array=w607) -> (size(s)=w605:i32)
        n204 = Format Into String(format string="Are you sure you want to delete \"%s\" and all %d callers?" ("message"), w606, w605) -> (resulting string=w603:string)  [unwired: 2 in, 1 out]
        n205 = Two Button Dialog(message=w603, 2:"Yes: Delete All" ("T button name (\"OK\")")) -> (T button?=w609:bool)  [unwired: 1 in]
        n206 = case shown="True" w609 {
          tunnel: w608 -> [w614 w628]
          tunnel: w612 -> [w615 w621]
          tunnel: [w614 w628] -> w610
          tunnel: [w615 w618] -> w611
          tunnel: [_ "Macro: Exit"] -> w602
          frame False {
          }
          frame True {
            n207 = Unbundle By Name(w628) -> ("State"=w626:string, "JKI SM out"=w622:refnum<class "JKI SM.lvclass">)
            n208 = call "Get VI Reference.vi"("error in (no error)"=w621, "JKI SM in"=w622) -> ("error out"=w623:errorcluster, "VI"=w616:refnum<vi>)  [unwired: 7 in, 1 out]
            n209 = call "Begin Undo Transaction.vi"("error in (no error)"=w623, "Action"="Delete State", "VI in"=w616) -> ("error out"=w620:errorcluster, "VI out"=w617:refnum<vi>)  [unwired: 7 in]
            n210 = call "Delete State.vi"("Delete Callers? (F: Only Delete Case Structure Frame)"=TRUE, "error in (no error)"=w620, "State Name"=w626, "JKI SM in"=w622) -> ("error out"=w619:errorcluster)  [unwired: 6 in, 1 out]
            n211 = call "End Undo Transaction.vi"("error in (no error)"=w619, "VI in"=w617) -> ("error out"=w618:errorcluster)  [unwired: 8 in, 1 out]
          }
        }
        n212 = call <vilib>:"Add State(s) to Queue__jki_lib_state_machine.vi"("State(s) in Front (\"\")"=w602, "State(s) in (\"\")"=w600) -> ("States Out"=w613:string)  [unwired: 13 in]
      }
      frame "New Category: 2" {
        # "Your code here.\n(You can make a copy of, or modify, this frame)"
        n213 = call <vilib>:"Add State(s) to Queue__jki_lib_state_machine.vi"("State(s) in (\"\")"=w632) -> ("States Out"=w631:string)  [unwired: 14 in]
      }
    }
  }
  "error out" <- w3
